vi "Method No Arguments.vi"(8 "error in (no error)":errorcluster, 11 "Mock In":refnum<class "Test Interface Mock.lvclass">) -> (0 "error out":errorcluster, 3 "Mock Out":refnum<class "Test Interface Mock.lvclass">)   [LabVIEW 2020, in "Test Interface Mock.lvclass"]
uses:
  Test Interface Mock.lvclass
  C:/git/astemes-lmock/source/Framework/Mock/LMock Mock.lvclass
  source/Framework/Mock/LMock Mock.lvclass
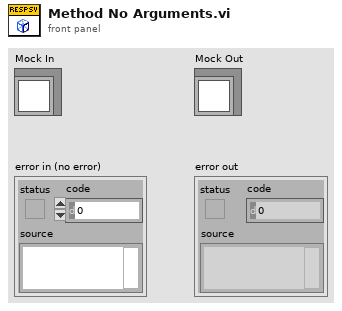
[diagram p1: front panel]
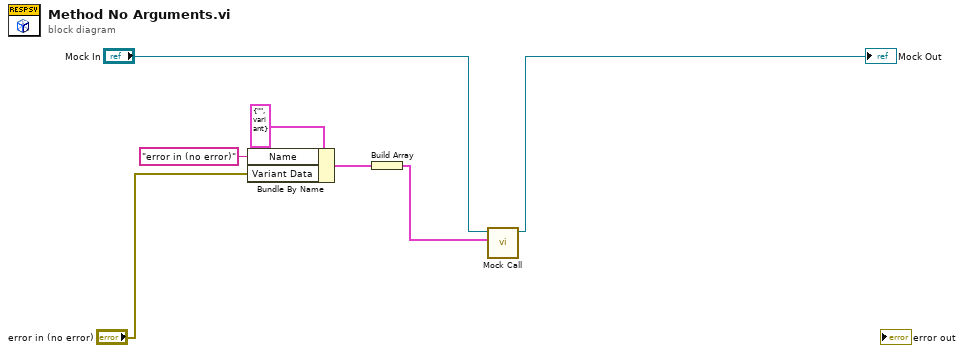
[diagram p0: block diagram]
diagram:
  n1 = Bundle By Name(cluster=cluster{"Name":string, "Variant Data":variant} {"Name"="", "Variant Data"=variant} ("element"), "Name"="error in (no error)", "Variant Data"="error in (no error)") -> (w2:cluster{"Name":string, "Variant Data":variant})
  n2 = Build Array(w2) -> (w1:cluster{"Name":string, "Variant Data":variant}[])
  n3 = call "Mock Call.vi"("Control Values"=w1, "Mock In"="Mock In") -> ("Mock Out"=→"Mock Out":refnum<class "Test Interface Mock.lvclass">)  [unwired: 8 in, 1 out]
